vi "Create Library if not Present.vi"(8 "error in":errorcluster, 9 "dest directory":path, 10 "project ref":refnum<vi>, 11 "virtual folder ref":refnum<vi>) -> (0 "error out":errorcluster, 3 "library refnum":refnum<vi>)   [LabVIEW 2021, in "Converter.lvlib"]
uses:
  Converter.lvlib
  Converter Reusables/Converter Reusables.lvlib
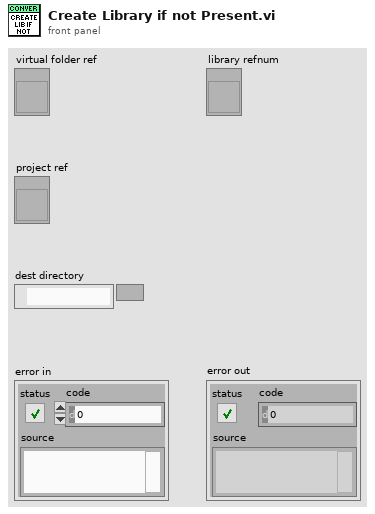
[diagram p1: front panel]
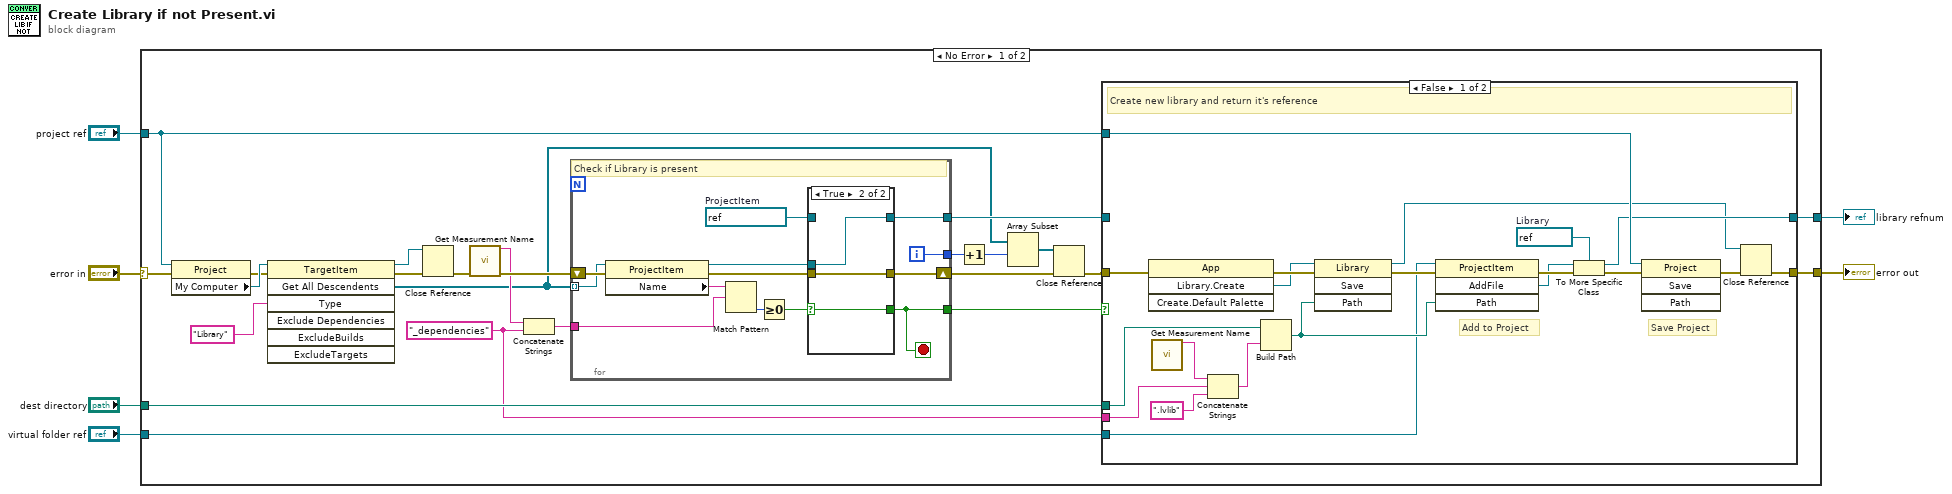
[diagram p0: block diagram]
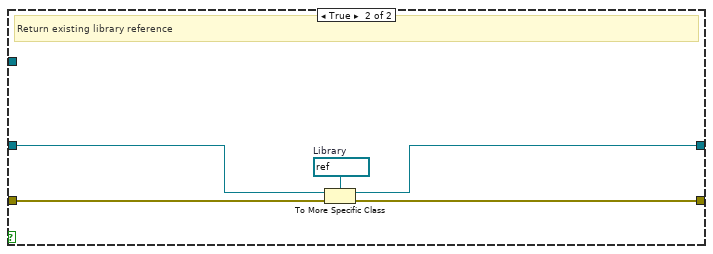
[diagram p2: hidden frame]
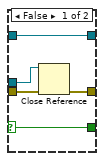
[diagram p3: hidden frame]
diagram:
  n1 = case shown="No Error" "error in" {
    selector: "error in" -> [w21 w77]
    tunnel: "dest directory" -> [w20 _]
    tunnel: "virtual folder ref" -> [w19 _]
    tunnel: "project ref" -> [w18 _]
    tunnel: [w17 w77] -> w2
    tunnel: [w15 _] -> w1
    frame No Error {
      w14 = "_dependencies" ("string")
      n2 = property class="Project"(reference=w18, error in=w21) -> (error out=w27:errorcluster, "My Computer"=w30:refnum<vi>)  [unwired: 1 out]
      n3 = invoke class="TargetItem" method="Get All Descendents"(reference=w30, error in=w27, "Type"="Library") -> (reference out=w28:refnum<vi>, error out=w29:errorcluster, "All Descendents"=w8:refnum<vi>[])  [unwired: 4 in, 4 out]
      n4 = Close Reference(reference=w28, error in (no error)=w29) -> (error out=w26:errorcluster)
      n5 = call "Get Measurement Name.vi"("error in"=w26) -> ("name out"=w24:string, "error out"=w25:errorcluster)  [unwired: 13 in]
      n6 = Concatenate Strings(w24, w14) -> (w23:string)
      n7 = for {
        tunnel: w8 -> [w67] mode=indexing
        tunnel: [w60] -> w16
        tunnel: w23 -> [w59]
        tunnel: [w58] -> w22
        shift-right: [w57] -> w12
        shift-left: w25 -> [w68]
        tunnel: [w56] -> w10
        i -> [w56]
        stop <- w58 stop-if-true
        w63 = refnum<vi> refnum  # ProjectItem
        # "Check if Library is present"
        n8 = property class="ProjectItem"(reference=w67, error in=w68) -> (reference out=w62:refnum<vi>, error out=w61:errorcluster, "Name"=w66:string)
        n9 = Match Pattern(string=w66, regular expression=w59) -> (offset past match=w65:i32)  [unwired: 1 in, 3 out]
        n10 = Greater Or Equal To 0?(x=w65) -> (x >= 0?=w64:bool)
        n11 = case shown="True" w64 {
          selector: w64 -> [w70 w75]
          tunnel: w62 -> [w71 w76]
          tunnel: [w73 w74] -> w57
          tunnel: [w72 w76] -> w60
          tunnel: w63 -> [w72 _]
          tunnel: [w70 w75] -> w58
          tunnel: w61 -> [w69 w74]
          frame False {
            n12 = Close Reference(reference=w71, error in (no error)=w69) -> (error out=w73:errorcluster)
          }
          frame True {
          }
        }
      }
      n13 = Increment(x=w10) -> (x+1=w9:i32)
      n14 = Array Subset(array=w8, index=w9) -> (w7:refnum<vi>[])  [unwired: 1 in]
      n15 = Close Reference(reference=w7, error in (no error)=w12) -> (error out=w11:errorcluster)
      n16 = case shown="False" w22 {
        tunnel: w11 -> [w50 w55]
        tunnel: w20 -> [w48 _]
        tunnel: w19 -> [w41 _]
        tunnel: w18 -> [w40 _]
        tunnel: [w34 w54] -> w17
        tunnel: w16 -> [_ w52]
        tunnel: [w35 w53] -> w15
        tunnel: w14 -> [w32 _]
        frame False {
          w36 = refnum<vi> refnum  # Library
          # "Save Project"
          # "Add to Project"
          # "Create new library and return it's reference"
          n17 = invoke class="App" method="Library.Create"(error in=w50) -> (error out=w49:errorcluster, "Create Library"=w45:refnum<vi>)  [unwired: 3 in, 2 out]
          n18 = call "Get Measurement Name.vi"() -> ("name out"=w47:string)  [unwired: 14 in, 1 out]
          n19 = Concatenate Strings(w47, w32, ".lvlib" ("string")) -> (w46:string)
          n20 = Build Path(base path=w48, name or relative path=w46) -> (appended path=w42:path)
          n21 = invoke class="Library" method="Save"(reference=w45, error in=w49, "Path"=w42) -> (reference out=w33:refnum<vi>, error out=w43:errorcluster)  [unwired: 1 in, 2 out]
          n22 = invoke class="ProjectItem" method="AddFile"(reference=w41, error in=w43, "Path"=w42) -> (error out=w44:errorcluster, "AddFile"=w37:refnum<vi>)  [unwired: 1 in, 2 out]
          n23 = To More Specific Class(target class=w36, reference=w37, error in=w44) -> (specific class reference=w35:refnum<vi>, error out=w38:errorcluster)
          n24 = invoke class="Project" method="Save"(reference=w40, error in=w38) -> (error out=w39:errorcluster)  [unwired: 2 in, 3 out]
          n25 = Close Reference(reference=w33, error in (no error)=w39) -> (error out=w34:errorcluster)
        }
        frame True {
          w51 = refnum<vi> refnum  # Library
          # "Return existing library reference"
          n26 = To More Specific Class(target class=w51, reference=w52, error in=w55) -> (specific class reference=w53:refnum<vi>, error out=w54:errorcluster)
        }
      }
    }
    frame Error {
    }
  }
  "error out" <- w2
  "library refnum" <- w1
